vi "HW XML Rx - Write.vi"(0 "String (in)":string, 1 "Use Octal Labels?":bool, 2 "Selected Channels":i32[](array[numeric]), 5 "formatting (NIVeriStandAdd-Ons)":enum16{"NIVeriStandAdd-Ons", "ni"}(ring), 7 "Parameter Array":T1[](array[typedef])) -> (4 "String (out)":string)   [LabVIEW 2023]
uses:
  Controls/Database_Array.ctl
  Controls/Encoding.ctl
  <userlib>/_OpenG.lib/array/array.llb/Remove Duplicates from 1D Array (I32)__ogtk.vi
  <userlib>/_OpenG.lib/array/array.llb/Filter 1D Array with Scalar (I32)__ogtk.vi
  <userlib>/_OpenG.lib/array/array.llb/Index 1D Array Elements (Variant)__ogtk.vi
  <userlib>/_OpenG.lib/array/array.llb/Remove Duplicates from 1D Array (U32)__ogtk.vi
  <userlib>/_OpenG.lib/array/array.llb/Filter 1D Array with Scalar (U32)__ogtk.vi
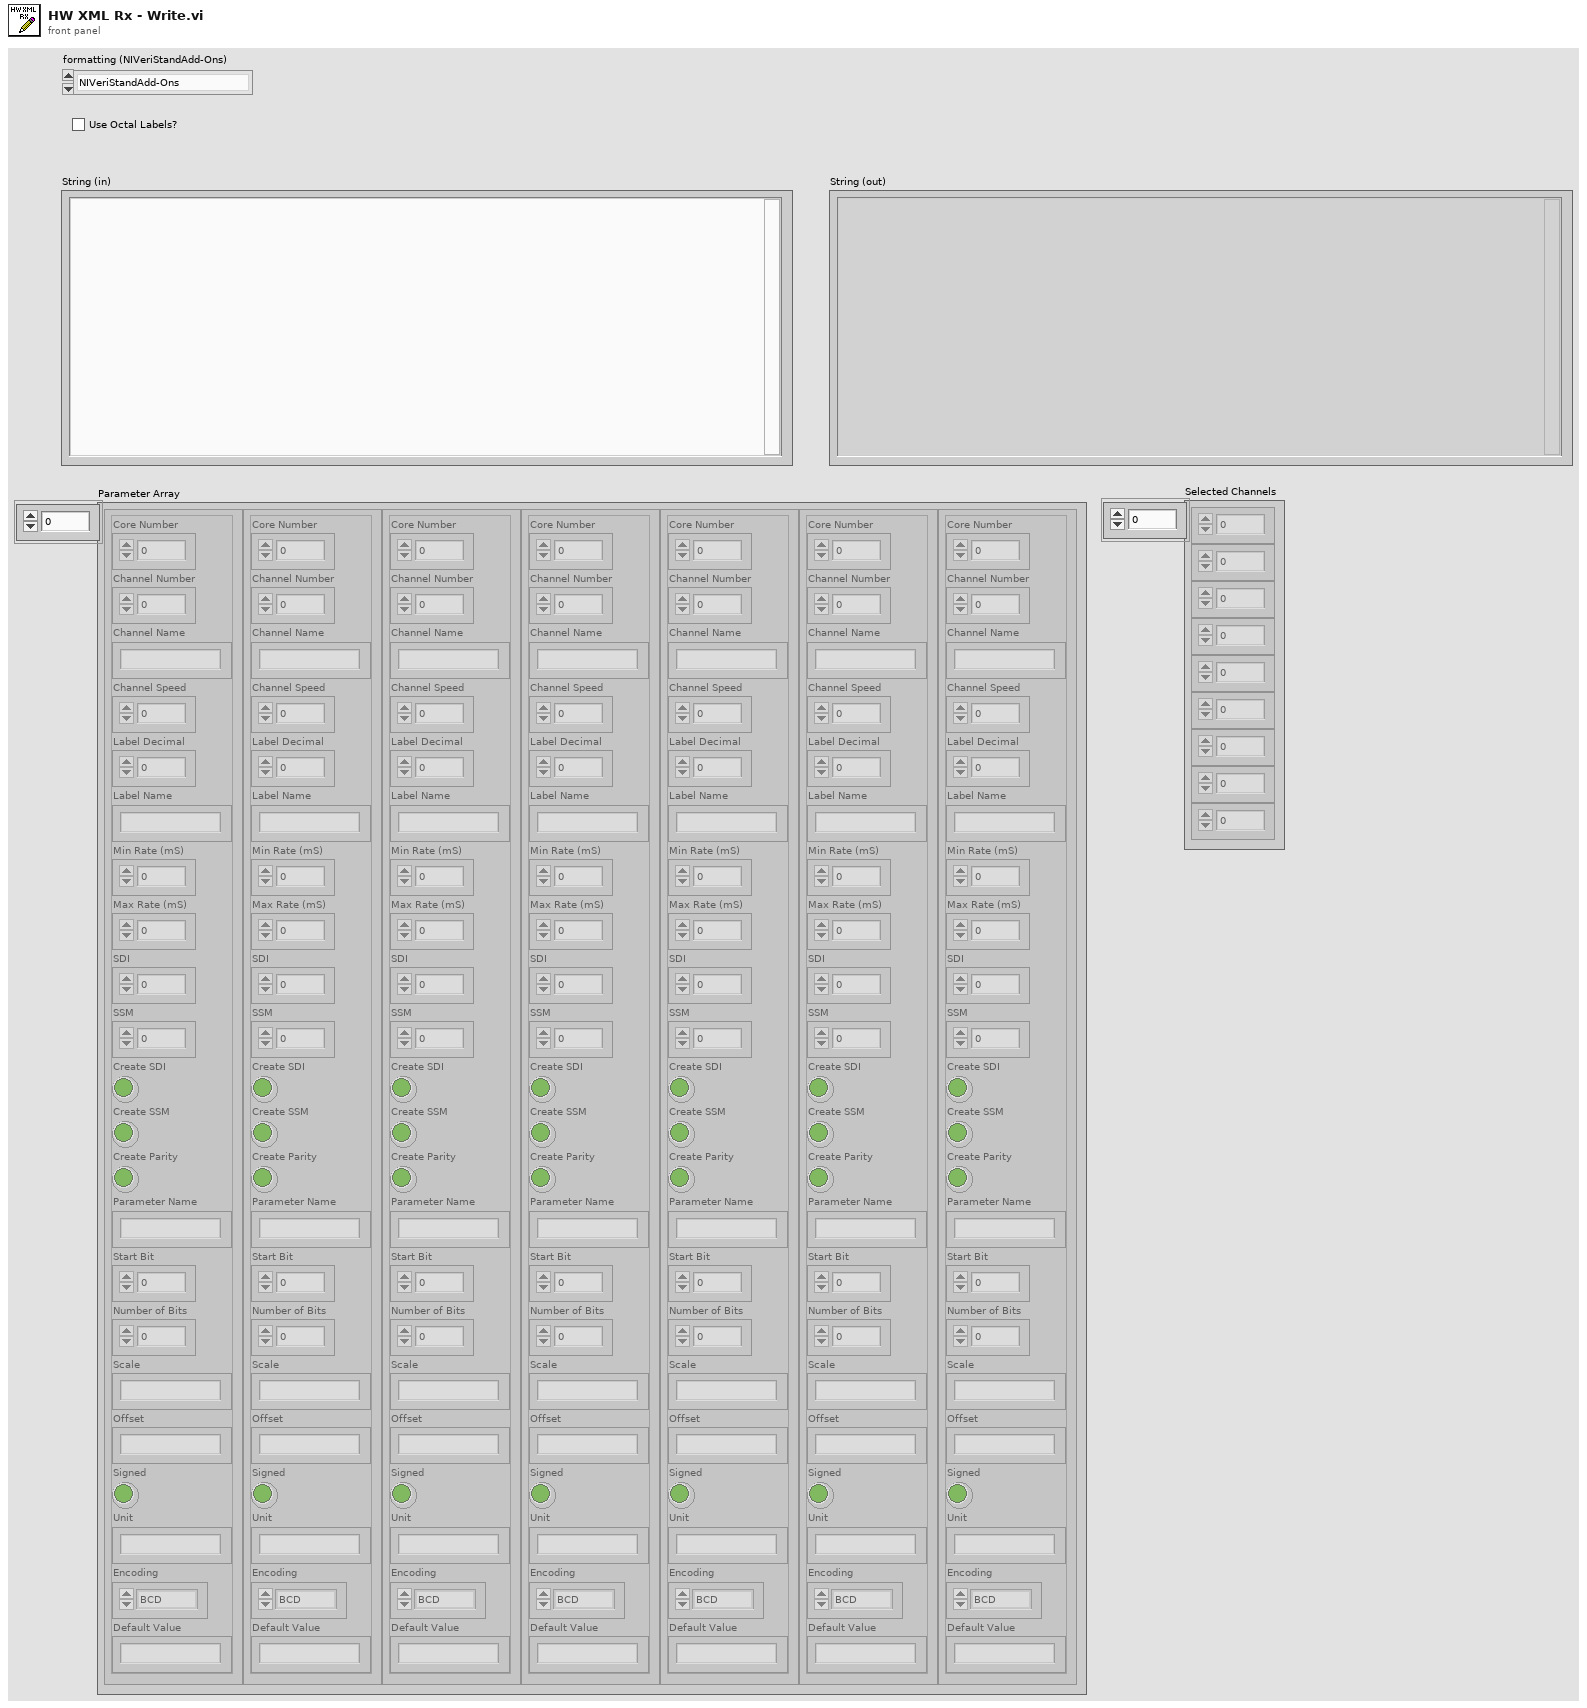
[diagram p1: front panel]
types:
  T1 = typedef "Database_Array.ctl" = cluster{"Core Number":i32, "Channel Number":i32, "Channel Name":string, "Channel Speed":i32, "Label Decimal":u32, "Label Name":string, "Min Rate (mS)":i32, "Max Rate (mS)":i32, "SDI":i32, "SSM":i32, "Create SDI":bool, "Create SSM":bool, "Create Parity":bool, "Parameter Name":string, "Start Bit":i32, "Number of Bits":i32, "Scale":string, "Offset":string, "Signed":bool, "Unit":string, "Encoding":T2, "Default Value":string}
  T2 = typedef "Encoding.ctl" = enum16{"BCD", "BNR", "Discrete"}
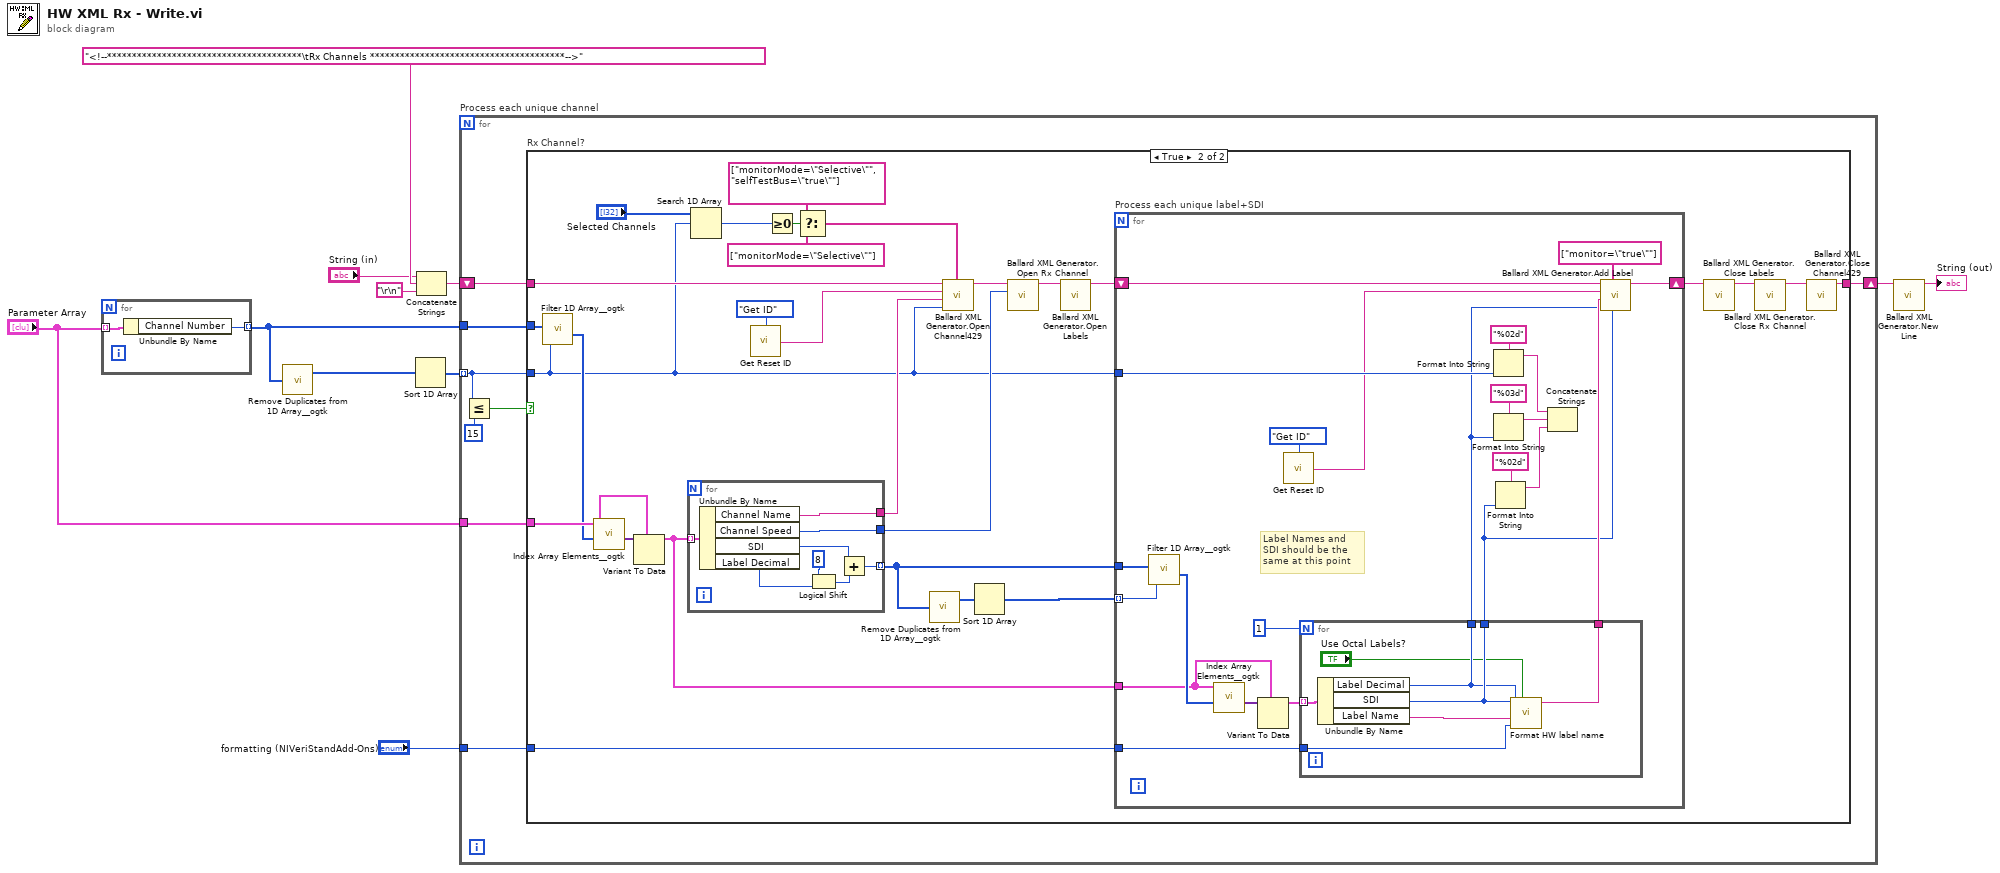
[diagram p0: block diagram]
diagram:
  n1 = for {
    tunnel: [w13] -> w4 mode=indexing
    tunnel: "Parameter Array" -> [w12] mode=indexing
    n2 = Unbundle By Name(w12) -> ("Channel Number"=w13:i32)
  }
  n3 = call-poly <userlib>:"Remove Duplicates from 1D Array__ogtk.vi"("Input Array"=w4) -> ("Output Array"=w10:i32[])  [unwired: 1 out]
  n4 = Sort 1D Array(array=w10) -> (sorted array=w11:i32[])
  n5 = Concatenate Strings("String (in)", "<!--***************************************\tRx Channels ***************************************-->", "\r\n") -> (w7:string)
  n6 = for "Process each unique channel" {
    tunnel: w11 -> [w19] mode=indexing
    shift-right: [w20] -> w2
    shift-left: w7 -> [w21]
    tunnel: w4 -> [w16]
    tunnel: "Parameter Array" -> [w15]
    tunnel: "formatting (NIVeriStandAdd-Ons)" -> [w14]
    n7 = Less Or Equal?(x=w19, y=15) -> (x <= y?=w18:bool)
    n8 = case "Rx Channel?" shown="True" w18 {
      tunnel: w21 -> [w22 w48]
      tunnel: [w22 w41] -> w20
      tunnel: w19 -> [_ w29]
      tunnel: w16 -> [_ w40]
      tunnel: w15 -> [_ w38]
      tunnel: w14 -> [_ w23]
      frame False {
      }
      frame True {
        n9 = call-poly <userlib>:"Filter 1D Array__ogtk.vi"("items to filter"=w29, "array"=w40) -> ("filtered item indices"=w36:i32[])  [unwired: 4 in, 1 out]
        n10 = call-poly <userlib>:"Index Array Elements__ogtk.vi"("indices"=w36, "array"=w38) -> ("elements"=w39:variant[])  [unwired: 9 in]
        n11 = Variant To Data(type=w38, Variant=w39) -> (data=w35:T1[])  [unwired: 1 in, 1 out]
        n12 = for {
          tunnel: w35 -> [w58] mode=indexing
          tunnel: [w57] -> w34
          tunnel: [w56] -> w33
          tunnel: [w52] -> w37 mode=indexing
          n13 = Unbundle By Name(w58) -> ("Channel Name"=w57:string, "Channel Speed"=w56:i32, "SDI"=w51:i32, "Label Decimal"=w53:u32)
          n14 = Logical Shift(y=i16 8, x=w53) -> (x << y=w55:u32)
          n15 = Add(x=w51, y=w55) -> (x+y=w52:u32)
        }
        n16 = Search 1D Array(1D array="Selected Channels", element=w29) -> (index of element=w28:i32)  [unwired: 1 in]
        n17 = call "Get Reset ID.vi"("Function"=enum16{"Get ID", "Reset ID"}."Get ID") -> ("ID"=w31:string)  [unwired: 14 in]
        n18 = Greater Or Equal To 0?(x=w28) -> (x >= 0?=w27:bool)
        n19 = Select(t=string[] ["monitorMode=\"Selective\"", "selfTestBus=\"true\""] ("other params"), s=w27, f=string[] ["monitorMode=\"Selective\""] ("other params")) -> (s? t:f=w24:string[])
        n20 = call-poly <userlib>:"Remove Duplicates from 1D Array__ogtk.vi"("Input Array"=w37) -> ("Output Array"=w50:u32[])  [unwired: 1 out]
        n21 = call "Ballard XML Generator.Open Channel429.vi"("other params"=w24, "hardware channel"=w29, "name"=w34, "id"=w31, "string in"=w48) -> ("string out"=w46:string)  [unwired: 6 in]
        n22 = Sort 1D Array(array=w50) -> (sorted array=w49:u32[])
        n23 = call "Ballard XML Generator.Open Rx Channel.vi"("speedKHz"=w33, "string in"=w46) -> ("string out"=w47:string)  [unwired: 9 in]
        n24 = call "Ballard XML Generator.Open Labels.vi"("string in"=w47) -> ("string out"=w45:string)  [unwired: 10 in]
        n25 = for "Process each unique label+SDI" {
          tunnel: w49 -> [w75] mode=indexing
          tunnel: w37 -> [w81]
          shift-right: [w78] -> w44
          shift-left: w45 -> [w79]
          tunnel: w29 -> [w74]
          tunnel: w35 -> [w69]
          tunnel: w23 -> [w59]
          # "Label Names and SDI should be the same at this point"
          n26 = call-poly <userlib>:"Filter 1D Array__ogtk.vi"("items to filter"=w75, "array"=w81) -> ("filtered item indices"=w71:i32[])  [unwired: 4 in, 1 out]
          n27 = call-poly <userlib>:"Index Array Elements__ogtk.vi"("indices"=w71, "array"=w69) -> ("elements"=w70:variant[])  [unwired: 9 in]
          n28 = Variant To Data(type=w69, Variant=w70) -> (data=w68:T1[])  [unwired: 1 in, 1 out]
          n29 = call "Get Reset ID.vi"("Function"=enum16{"Get ID", "Reset ID"}."Get ID") -> ("ID"=w60:string)  [unwired: 14 in]
          n30 = for {
            N: 1 -> [_]
            tunnel: w68 -> [w88] mode=indexing
            tunnel: [w87] -> w67
            tunnel: [w84] -> w66
            tunnel: [w85] -> w62
            tunnel: w59 -> [w83]
            n31 = Unbundle By Name(w88) -> ("Label Decimal"=w84:u32, "SDI"=w85:i32, "Label Name"=w86:string)
            n32 = call "Format HW label name.vi"("Use Octal Channel Names?"="Use Octal Labels?", "formatting"=w83, "Label Name in"=w86, "SDI"=w85, "Label Decimal"=w84) -> ("Label Name out"=w87:string)  [unwired: 6 in]
          }
          n33 = Format Into String(format string="%02d", w74) -> (resulting string=w73:string)  [unwired: 2 in, 1 out]
          n34 = Format Into String(format string="%03d", w66) -> (resulting string=w72:string)  [unwired: 2 in, 1 out]
          n35 = Format Into String(format string="%02d", w62) -> (resulting string=w63:string)  [unwired: 2 in, 1 out]
          n36 = Concatenate Strings(w73, w72, w63) -> ()  [unwired: 1 out]
          n37 = call "Ballard XML Generator.Add Label.vi"("SDI"=w62, "other params"=string[] ["monitor=\"true\""], "label decimal"=w66, "name"=w67, "id"=w60, "string in"=w79) -> ("string out"=w78:string)  [unwired: 5 in]
        }
        n38 = call "Ballard XML Generator.Close Labels.vi"("string in"=w44) -> ("string out"=w43:string)  [unwired: 10 in]
        n39 = call "Ballard XML Generator.Close Rx Channel.vi"("string in"=w43) -> ("string out"=w42:string)  [unwired: 10 in]
        n40 = call "Ballard XML Generator.Close Channel429.vi"("string in"=w42) -> ("string out"=w41:string)  [unwired: 10 in]
      }
    }
  }
  n41 = call "Ballard XML Generator.New Line.vi"("string in"=w2) -> ("string out"=→"String (out)":string)  [unwired: 10 in]
